vi "Serial_test_Query.vi"() -> ()   [LabVIEW 2026]
panel:
  out "Reply":string
  in  "ESP32_Data":refnum<visa-resource-name>="COM20"
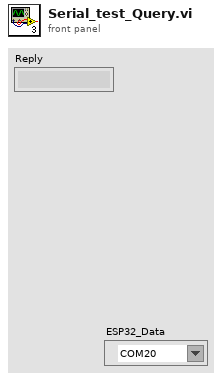
[diagram p1: front panel]
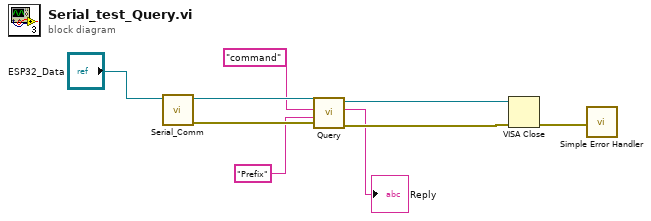
[diagram p0: block diagram]
diagram:
  n1 = call "Serial_Comm.vi"("ESP32_Data"="ESP32_Data") -> ("Roll_result"=w7:refnum<visa-resource-name>, "error out"=w6:errorcluster)  [unwired: 8 in]
  n2 = call "Query.vi"("error in (no error)"=w6, "Prefix"="Prefix", "command"="command", "VISA Res IN"=w7) -> ("error out"=w4:errorcluster, "Reply"=→"Reply":string, "VISA Res OUT"=w5:refnum<visa-resource-name>)  [unwired: 5 in]
  n3 = VISA Close(VISA resource name=w5, error in (no error)=w4) -> (error out=w8:errorcluster)
  n4 = call <vilib>:"Simple Error Handler.vi"("error in (no error)"=w8) -> ()  [unwired: 4 in, 5 out]
